vi "Client.vi"() -> ()   [LabVIEW 2021]
doc: "This VI acts as a client for an incoming websockets connection. Receives/sends string data to the connected client."
uses:
  StatusCode.ctl
  LV WebSockets.lvlib
panel:
  in  "TLS server hostname":string="lvtls.example"
  out "Status Code":T1=1000 items=["Normal Closure"=1000, "Going Away"=1001, "Protocol Error"=1002, "Wrong Data Type"=1003, "Reserved 1004"=1004, "Reserved 1005"=1005, "Reserved 1006"=1006, "Non Consistent Data Type"=1007, "Policy Violation"=1008, "Message Too Big"=1009, "Extensions Negotiation Error"=1010, "Unexpected Condition"=1011, "Reserved 1015"=1015]
  out "Close Reason":string
  in  "WS URI":string="ws://localhost:6123/resource/name"
  out "Resource Name":string
  out "HTTP Headers":variant
  in  "Stop":bool
  out "Received Data":string
  in  "Send":bool
  in  "Data":string
  # "WebSockets Example Client"
  # "This VI is a simple example of sending/receiving data using WebSockets.\nIt opens a WebSockets connection on Port 6123 and\nthen displays incoming string data. Strings can also be sent back to the client.\nInstructions for use:\n1) Run the SingleConnection.vi VI\n2) Set a suitable websocket URI including a resource name matching the one defined on the server and the right protocol (ws or wss) matching the one adopted by the server\n2a) TLS server hostname: if you are testing the TLS secured communication with the LV-WebSockets server via self signed cetificates set this control to \"lvtls.example\" (default)\n2b) TLS server hostname: if you want to test any other TLS secured WebSocket server set this control to the server hostname. For example if you are testing the Postman Echo service wss://ws.postman-echo.com/raw set this control to \"ws.postman-echo.com\"\n3) Quickly run this VI"
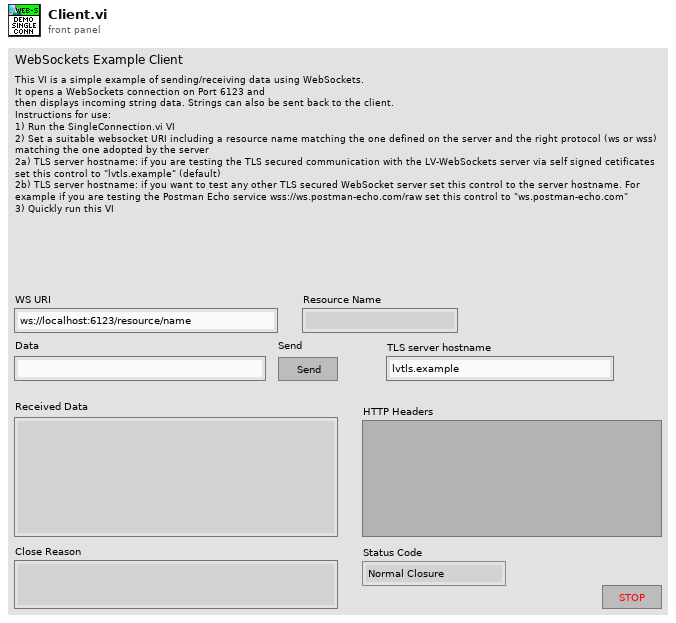
[diagram p1: front panel]
types:
  T1 = typedef "LV WebSockets.lvlib/StatusCode.ctl" = u16
  T2 = typedef "LV WebSockets.lvlib/Opcode.ctl" = enum8{"Continuation Frame", "Text Frame", "Binary Frame", "Reserved 3", "Reserved 4", "Reserved 5", "Reserved 6", "Reserved 7", "Connection Close", "Ping", "Pong", "Reserved B", "Reserved C", "Reserved D", "Reserved F"}
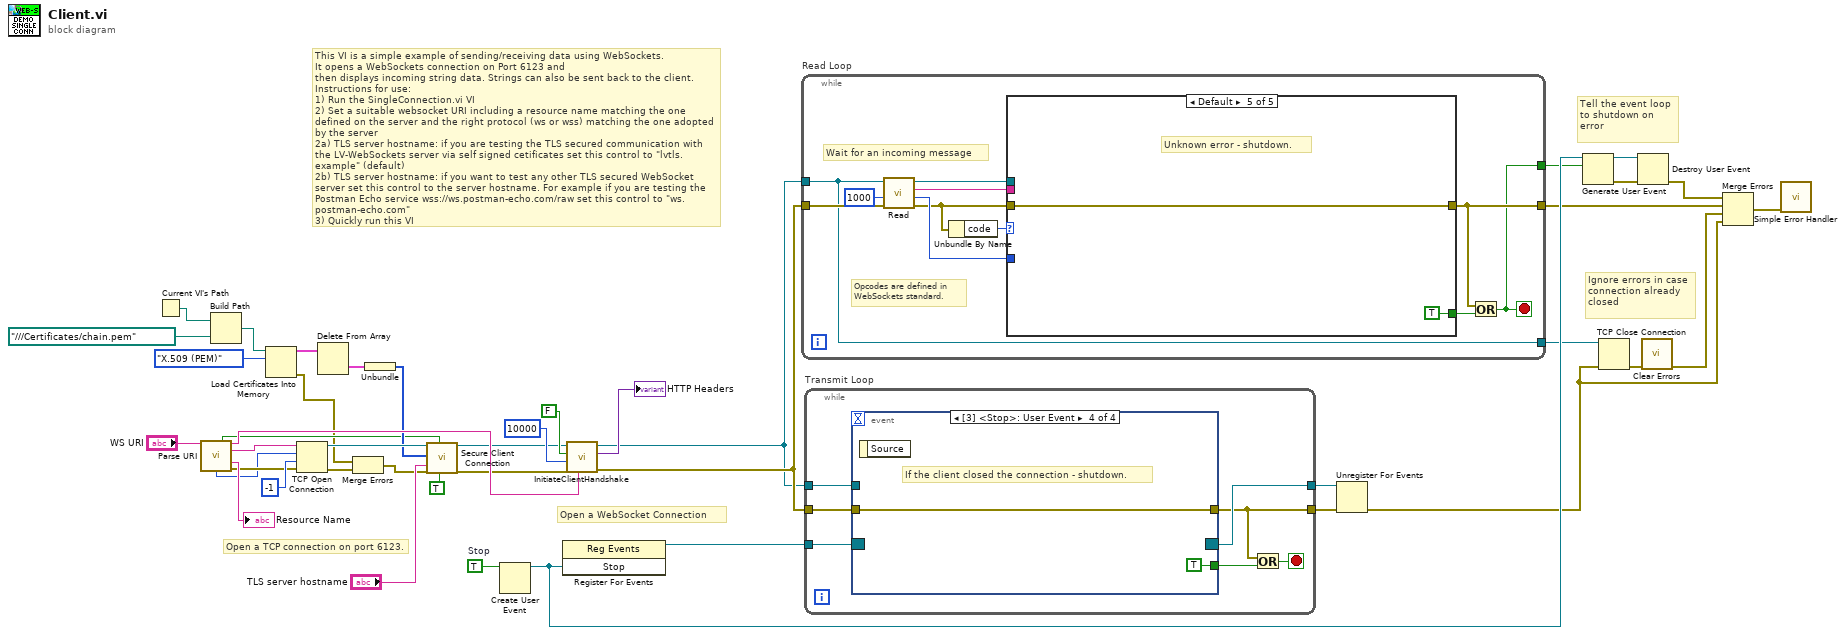
[diagram p0: block diagram]
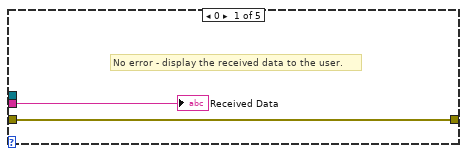
[diagram p2: hidden frame]
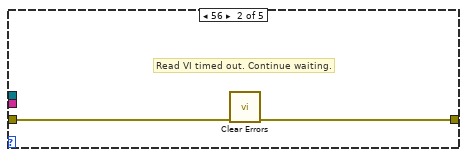
[diagram p3: hidden frame]
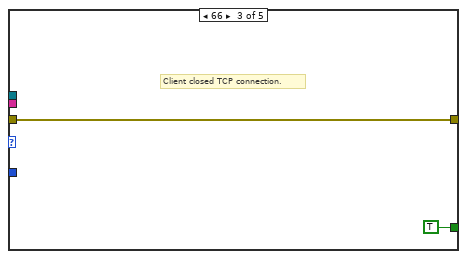
[diagram p4: hidden frame]
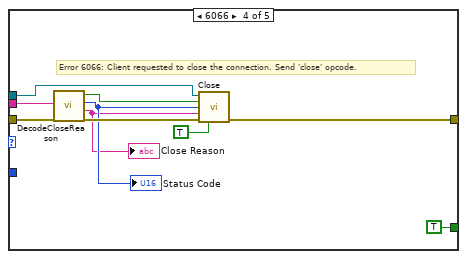
[diagram p5: hidden frame]
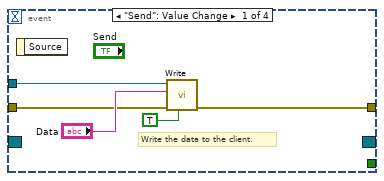
[diagram p6: hidden frame]
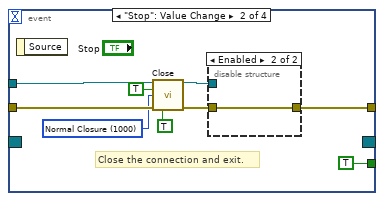
[diagram p7: hidden frame]
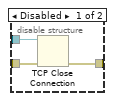
[diagram p8: hidden frame]
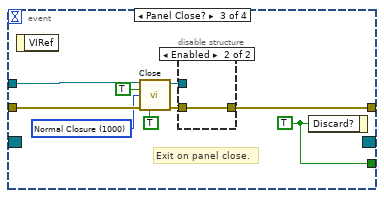
[diagram p9: hidden frame]
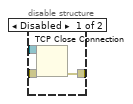
[diagram p10: hidden frame]
diagram:
  w41 = TRUE  # Stop
  # "Ignore errors in case\nconnection already\nclosed"
  # "Tell the event loop to shutdown on error"
  # "This VI is a simple example of sending/receiving data using WebSockets.\nIt opens a WebSockets connection on Port 6123 and\nthen displays incoming string data. Strings can also be sent back to the client.\nInstructions for use:\n1) Run the SingleConnection.vi VI\n2) Set a suitable websocket URI including a resource name matching the one defined on the server and the right protocol (ws or wss) matching the one adopted by the server\n2a) TLS server hostname: if you are testing the TLS secured communication with the LV-WebSockets server via self signed cetificates set this control to \"lvtls.example\" (default)\n2b) TLS server hostname: if you want to test any other TLS secured WebSocket server set this control to the server hostname. For example if you are testing the Postman Echo service wss://ws.postman-echo.com/raw set this control to \"ws.postman-echo.com\"\n3) Quickly run this VI"
  # "Open a WebSocket Connection"
  # "Open a TCP connection on port 6123."
  n1 = Current VI's Path() -> (path=w6:path)
  n2 = call "Parse URI.vi"("URI"="WS URI") -> ("Secure"=w7:bool, "URI Out"=w27:string, "Hostname"=w26:string, "Resource Name"=→"Resource Name":string, "Port"=w22:u16, "error out"=w24:errorcluster)  [unwired: 7 in, 2 out]
  n3 = Build Path(base path=w6, name or relative path=path "../../../Certificates/chain.pem" ("cert chain")) -> (appended path=w16:path)
  n4 = Load Certificates Into Memory(10:enum32{"X.509 (PEM)"}."X.509 (PEM)" ("format"), 11:w16) -> (0:w4:errorcluster, 3:w9:cluster{"certificate":u8[]}[])  [unwired: 1 in]
  n5 = TCP Open Connection(address=w26, remote port or service name=w22, timeout ms (60000)=-1 ("timeout ms (25000)"), error in (no error)=w24) -> (connection ID=w12:refnum<k5>, error out=w15:errorcluster)  [unwired: 1 in]
  n6 = Delete From Array(array=w9) -> (deleted portion=w10:cluster{"certificate":u8[]})  [unwired: 2 in, 1 out]
  n7 = Merge Errors(w4, w15) -> (w5:errorcluster)
  n8 = Unbundle(w10) -> ("certificate"=w8:u8[])
  n9 = call "Secure Client Connection.vi"("TCP connection"=w12, "certificate"=w8, "server hostname"="TLS server hostname", "error in"=w5, "Secure the Connection (T)"=w7, "load OS trusted CAs?"=TRUE) -> ("TCP connection out"=w13:refnum<k5>, "error out"=w14:errorcluster)  [unwired: 11 in, 1 out]
  n10 = Create User Event(user event datatype=w41) -> (user event=w39:refnum<user-event>)  [unwired: 1 in, 1 out]
  n11 = register-events(w39) -> (reference out=w42:refnum<event-registration>)  [unwired: 2 in, 1 out]
  n12 = call "InitiateClientHandshake.vi"("WS URI"=w27, "error in (no error)"=w14, "timeout ms (5000)"=10000 ("timeout ms (25000)"), "Relative URI Request (F)"=FALSE, "WebSocket Connection in"=w13) -> ("error out"=w31:errorcluster, "Return Headers Out"=→"HTTP Headers":variant, "WebSocket Connection out"=w3:refnum<k5>)  [unwired: 4 in]
  n13 = while "Read Loop" {
    tunnel: w3 -> [w44]
    tunnel: [w45] -> w38
    tunnel: [w47] -> w30
    tunnel: w31 -> [w48]
    tunnel: [w44] -> w19
    stop <- w45 stop-if-true
    # "Wait for an incoming message"
    # "Opcodes are defined in\nWebSockets standard."
    n14 = call "Read.vi"("error in (no error)"=w48, "timeout ms (5000)"=1000 ("timeout ms (25000)"), "WebSocket Connection in"=w44) -> ("error out"=w49:errorcluster, "Opcode out"=w50:T2, "Data"=w52:string, "WebSocket Connection out"=w51:refnum<k5>)  [unwired: 5 in]
    n15 = Unbundle By Name(w49) -> ("code"=w53:i32)
    n16 = case shown="Default" w53 {
      tunnel: w52 -> [w56 _ _ w65 _]
      tunnel: [_ _ TRUE TRUE TRUE] -> w46
      tunnel: w51 -> [_ _ _ w69 _]
      tunnel: w50 -> [_ _ _ _ _]
      tunnel: w49 -> [w55 w58 w59 w67 w70]
      tunnel: [w55 w57 w59 w66 w70] -> w47
      frame 0 {
        # "No error - display the received data to the user."
        "Received Data" <- w56
      }
      frame 56 {
        # "Read VI timed out. Continue waiting."
        n17 = call <vilib>:"Clear Errors.vi"("error in (no error)"=w58) -> ("error out"=w57:errorcluster)  [unwired: 5 in, 1 out]
      }
      frame 66 {
        # "Client closed TCP connection."
      }
      frame 6066 {
        # "Error 6066: Client requested to close the connection. Send 'close' opcode."
        n18 = call "DecodeCloseReason.vi"("Data"=w65) -> ("Reason"=w61:string, "Status Code"=w63:T1, "Close Reason Given"=w64:bool)  [unwired: 8 in]
        "Close Reason" <- w61
        "Status Code" <- w63
        n19 = call "Close.vi"("WebSocket Connection in"=w69, "Send Reason (F)"=w64, "Status Code"=w63, "Reason"=w61, "error in (no error)"=w67, "Mask payload?"=TRUE) -> ("error out"=w66:errorcluster)  [unwired: 8 in, 1 out]
      }
      frame Default {
        # "Unknown error - shutdown."
      }
    }
    n20 = Or(x=w47, y=w46) -> (x .or. y?=w45:bool)
  }
  n21 = while "Transmit Loop" {
    tunnel: w3 -> [w78]
    tunnel: w42 -> [w77]
    tunnel: [w76] -> w40
    tunnel: [w72] -> w32
    tunnel: w31 -> [w75]
    stop <- w73 stop-if-true
    n22 = event shown="[3] <Stop>: User Event" {
      selector: w77 -> [_ _ _ _]
      dyn-events: [_ _ _ _] -> w76
      timeout: _ -> [_ _ _ _]
      tunnel: w78 -> [w83 w91 w105 _]
      tunnel: [_ TRUE w103 TRUE] -> w74
      tunnel: [w80 w89 w101 w110] -> w72
      tunnel: w75 -> [w81 w87 w100 w110]
      event "Send": Value Change {
        # "Write the data to the client."
        n23 = event-data() -> ()  [unwired: 1 in, 1 out]
        n24 = call "Write.vi"("Mask payload?"=TRUE, "error in (no error)"=w81, "Data"="Data", "WebSocket Connection in"=w83) -> ("error out"=w80:errorcluster)  [unwired: 6 in, 1 out]
      }
      event "Stop": Value Change {
        w85 = T1 1000 items=["Normal Closure"=1000, "Going Away"=1001, "Protocol Error"=1002, "Wrong Data Type"=1003, "Reserved 1004"=1004, "Reserved 1005"=1005, "Reserved 1006"=1006, "Non Consistent Data Type"=1007, "Policy Violation"=1008, "Message Too Big"=1009, "Extensions Negotiation Error"=1010, "Unexpected Condition"=1011, "Reserved 1015"=1015] ("Status Code")
        # "Close the connection and exit."
        n25 = event-data() -> ()  [unwired: 1 in, 1 out]
        n26 = call "Close.vi"("WebSocket Connection in"=w91, "Send Reason (F)"=TRUE, "Status Code"=w85, "error in (no error)"=w87, "Mask payload?"=TRUE) -> ("WebSocket Connection in"=w90:refnum<k5>, "error out"=w88:errorcluster)  [unwired: 9 in]
        n27 = disable-structure shown="Enabled" {
          disable-tunnel: w90 -> [w95 _]
          disable-tunnel: [w94 w96] -> w89
          disable-tunnel: w88 -> [w93 w96]
          frame Disabled {
            n28 = TCP Close Connection(connection ID=w95, error in (no error)=w93) -> (error out=w94:errorcluster)  [unwired: 1 in, 1 out]
          }
          frame Enabled {
          }
        }
      }
      event Panel Close? {
        w98 = T1 1000 items=["Normal Closure"=1000, "Going Away"=1001, "Protocol Error"=1002, "Wrong Data Type"=1003, "Reserved 1004"=1004, "Reserved 1005"=1005, "Reserved 1006"=1006, "Non Consistent Data Type"=1007, "Policy Violation"=1008, "Message Too Big"=1009, "Extensions Negotiation Error"=1010, "Unexpected Condition"=1011, "Reserved 1015"=1015] ("Status Code")
        w103 = TRUE ("Discard?")
        # "Exit on panel close."
        n29 = event-data() -> ()  [unwired: 1 in, 1 out]
        n30 = call "Close.vi"("WebSocket Connection in"=w105, "Send Reason (F)"=TRUE, "Status Code"=w98, "error in (no error)"=w100, "Mask payload?"=TRUE) -> ("WebSocket Connection in"=w104:refnum<k5>, "error out"=w102:errorcluster)  [unwired: 9 in]
        n31 = disable-structure shown="Enabled" {
          disable-tunnel: w104 -> [w108 _]
          disable-tunnel: w102 -> [w107 w109]
          disable-tunnel: [w106 w109] -> w101
          frame Disabled {
            n32 = TCP Close Connection(connection ID=w108, error in (no error)=w107) -> (error out=w106:errorcluster)  [unwired: 1 in, 1 out]
          }
          frame Enabled {
          }
        }
        n33 = event-data("Discard?"=w103) -> ()  [unwired: 1 in, 1 out]
      }
      event User Event {
        # "If the client closed the connection - shutdown."
        n34 = event-data() -> ()  [unwired: 1 in, 1 out]
      }
    }
    n35 = Or(x=w72, y=w74) -> (x .or. y?=w73:bool)
  }
  n36 = Unregister For Events(event registration refnum=w40, error in=w32) -> (error out=w20:errorcluster)
  n37 = Generate User Event(user event=w39, event data cluster=w38) -> (user event out=w37:refnum<user-event>, error out=w36:errorcluster)  [unwired: 2 in]
  n38 = TCP Close Connection(connection ID=w19, error in (no error)=w20) -> (error out=w29:errorcluster)  [unwired: 1 in, 1 out]
  n39 = Destroy User Event(user event=w37, error in=w36) -> (error out=w35:errorcluster)
  n40 = call <vilib>:"Clear Errors.vi"("error in (no error)"=w29) -> ("error out"=w21:errorcluster)  [unwired: 5 in, 1 out]
  n41 = Merge Errors(w35, w30, w21, w20) -> (w2:errorcluster)
  n42 = call <vilib>:"Simple Error Handler.vi"("error in (no error)"=w2) -> ()  [unwired: 4 in, 5 out]
